vi "Run.vi"(8 "error in (no error)":errorcluster, 10 "UI Refs":T1, 11 "F18 Blowdown":refnum<class "F18 Blowdown.lvclass">) -> (0 "error out":errorcluster, 3 "F18 Blowdown out":refnum<class "F18 Blowdown.lvclass">)   [LabVIEW 2025, in "F18 Blowdown.lvlib" / "F18 Blowdown.lvclass"]
uses:
  F18 Blowdown.lvclass
  Users/Public/Documents/Sandia National Labs/TSS Plugin/Tests/XY Plotter.lvlibp/XY  Plotter/XY Plotter.lvclass
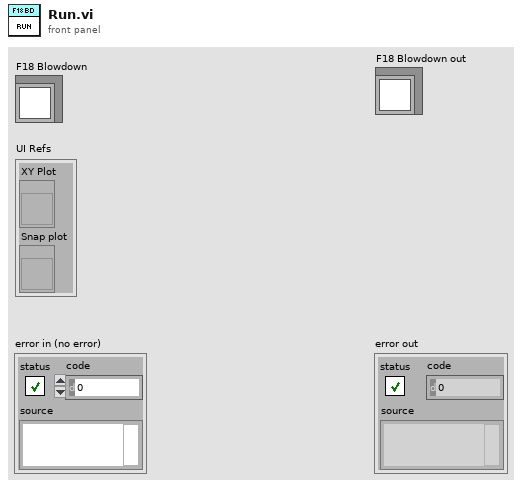
[diagram p1: front panel]
types:
  T1 = cluster{"XY Plot":refnum<vi>, "Snap plot":refnum<vi>}
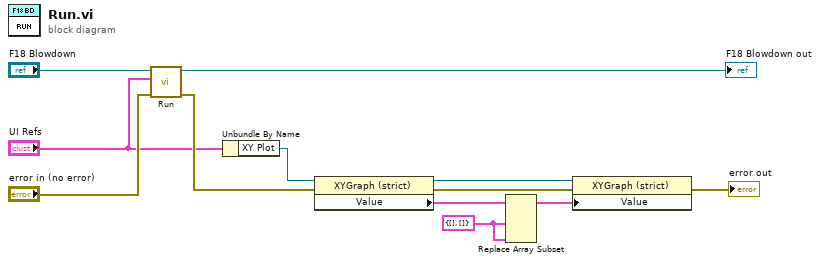
[diagram p0: block diagram]
diagram:
  w11 = cluster{"Wavenumber":dbl[], "Data":dbl[]} {"Wavenumber"=[], "Data"=[]} ("Spectrum")
  n1 = call-parent "Run.vi"("error in (no error)"="error in (no error)", "UI Refs"="UI Refs", "XY Plotter"="F18 Blowdown") -> ("error out"=w6:errorcluster, "XY Plotter out"=→"F18 Blowdown out":refnum<class "F18 Blowdown.lvclass">)  [unwired: 7 in]
  n2 = Unbundle By Name("UI Refs") -> ("XY Plot"=w1:refnum<vi>)
  n3 = property class="XYGraph (strict)"(reference=w1, error in=w6) -> (reference out=w9:refnum<vi>, error out=w5:errorcluster, "Value"=w10:cluster{"Wavenumber":dbl[], "Data":dbl[]}[])
  n4 = Replace Array Subset(array=w10, new element #1=w11, new element #2=w11) -> (w8:cluster{"Wavenumber":dbl[], "Data":dbl[]}[])  [unwired: 2 in]
  n5 = property class="XYGraph (strict)"(reference=w9, error in=w5, "Value"=w8) -> (error out=→"error out":errorcluster)  [unwired: 1 out]
